vi "Send MCP request (headers).vi"(6 "timeout (10000)":i32=10000, 8 "error in (no error)":errorcluster, 9 "request":string, 10 "request headers":string, 11 "url":string="http://localhost:36987/mcp/server") -> (0 "error out":errorcluster, 1 "response":string, 2 "headers":string, 3 "status code":i32)   [LabVIEW 2020, in "MCP Server tests.lvlib"]
doc: "Test helper. POSTs request to url with the request headers given one per line as Name: value, and returns the numeric HTTP status code, the raw response headers and the response body.\n\nNo header is added on its own, so Content-Type has to be one of the lines. status code is parsed from the status line at the start of headers; 0 when none was received."
uses:
  MCP Server tests.lvlib
  <vilib>/httpClient/POSTBuffer.vi
  <vilib>/httpClient/LabVIEWHTTPClient.lvlib
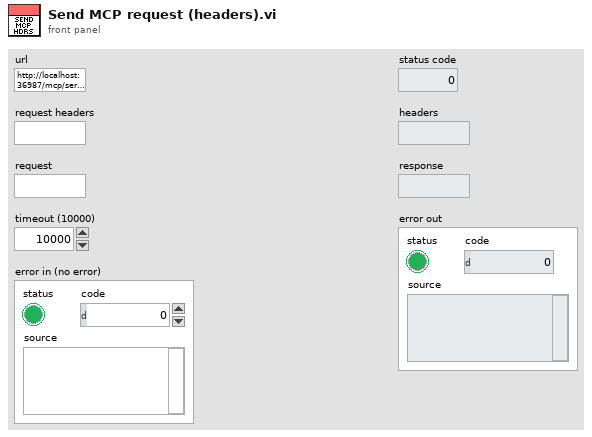
[diagram p1: front panel]
types:
  T1 = typedef "LabVIEWHTTPClient.lvlib/ClientHandle.ctl" = refnum<k1>
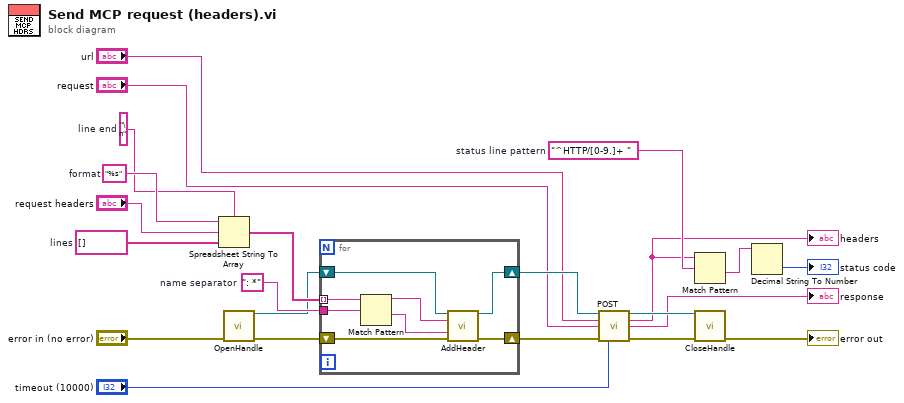
[diagram p0: block diagram]
diagram:
  w6 = "^HTTP/[0-9.]+ "  # status line pattern
  w16 = ": *"  # name separator
  w20 = string[] []  # lines
  w19 = "\n"  # line end
  w22 = "%s"  # format
  n1 = Spreadsheet String To Array(delimiter (Tab)=w19, format string=w22, spreadsheet string="request headers", array type (2D Dbl)=w20) -> (array=w17:string[])
  n2 = call <vilib>:"OpenHandle.vi"("error in (no error)"="error in (no error)") -> ("client handle out"=w15:T1, "error out"=w14:errorcluster)  [unwired: 13 in]
  n3 = for {
    tunnel: w17 -> [w30] mode=indexing
    tunnel: w16 -> [w29]
    shift-right: [w26] -> w13
    shift-left: w15 -> [w25]
    shift-right: [w24] -> w10
    shift-left: w14 -> [w23]
    n4 = Match Pattern(string=w30, regular expression=w29) -> (before substring=w28:string, after substring=w27:string)  [unwired: 1 in, 2 out]
    n5 = call <vilib>:"AddHeader.vi"("client handle"=w25, "header"=w28, "value"=w27, "error in (no error)"=w23) -> ("client handle out"=w26:T1, "error out"=w24:errorcluster)  [unwired: 10 in]
  }
  n6 = call-poly <vilib>:"POST.vi"("client handle"=w13, "url"="url", "buffer"="request", "error in (no error)"=w10, "timeout (10000)"="timeout (10000)") -> ("client handle out"=w8:T1, "headers"=w3:string, "body"=→"response":string, "error out"=w7:errorcluster)  [unwired: 7 in]
  "headers" <- w3
  n7 = Match Pattern(string=w3, regular expression=w6) -> (after substring=w5:string)  [unwired: 1 in, 3 out]
  n8 = call <vilib>:"CloseHandle.vi"("client handle"=w8, "error in (no error)"=w7) -> ("error out"=→"error out":errorcluster)  [unwired: 13 in]
  n9 = Decimal String To Number(string=w5) -> (number=→"status code":i32)  [unwired: 2 in, 1 out]
